vi "set RBW or VBW.vi"(6 "BW Auto?":bool, 8 "error in (no error)":errorcluster, 9 "BW Type":T1, 10 "BW Value (Hz)":dbl format="%#_6p", 11 "Interface_Spectrum in":refnum<class "Interface_Spectrum.lvclass">) -> (0 "error out":errorcluster, 3 "Interface_Spectrum out":refnum<class "Interface_Spectrum.lvclass">)   [LabVIEW 2023, in "Spectrum Analyzer.lvlib" / "Interface_Spectrum.lvclass"]
doc: "[RBW Setting]\n* For FSV-40\nParameters:\n<Bandwidth> refer to data sheet\n *RST: (AUTO is set to ON)\nExample:\n BAND 1 MHz\n Sets the resolution bandwidth to 1 MHz\n\n[VBW Setting]\n* For FSV-40\nParameters:\n<Bandwidth> refer to data sheet\n*RST: (AUTO is set to ON)\nExample: BAND:VID 10 kHz"
uses:
  Interface_Spectrum.lvclass
  TYPE DEFINITION/TYPE RBW and VBW Select.ctl
  Spectrum Analyzer.lvlib
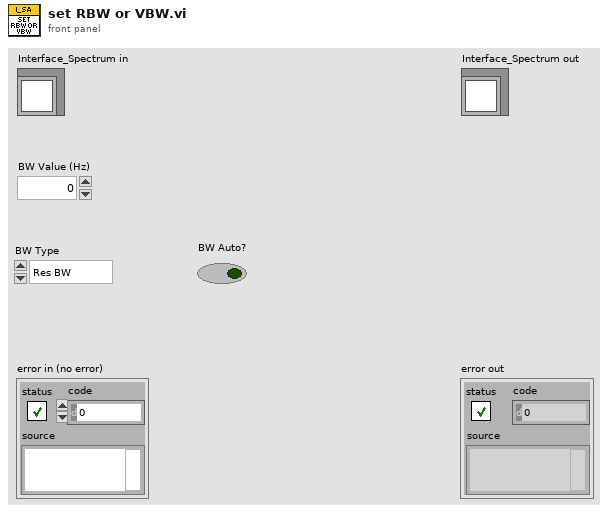
[diagram p1: front panel]
types:
  T1 = typedef "Spectrum Analyzer.lvlib/TYPE RBW and VBW Select.ctl" = enum16{"Res BW", "Video BW"}
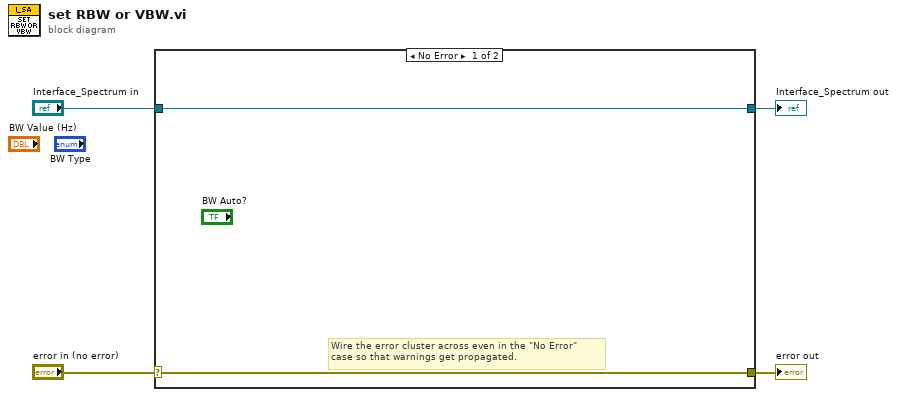
[diagram p0: block diagram]
diagram:
  n1 = case shown="No Error" "error in (no error)" {
    selector: "error in (no error)" -> [w5 w8]
    tunnel: [w5 w8] -> w3
    tunnel: [w6 w7] -> w1
    tunnel: "Interface_Spectrum in" -> [w6 w7]
    frame No Error {
      # "Wire the error cluster across even in the \"No Error\"\ncase so that warnings get propagated."
    }
    frame Error {
    }
  }
  "error out" <- w3
  "Interface_Spectrum out" <- w1
